vi "OwnCompat20261012_Native_GetRootDiagram.vi"() -> ()   [LabVIEW 2024]
panel:
  out "error out":errorcluster caption="错误输出"
  out "diagram_id":u32
  in  "diagram_id type":u32
  in  "target_path":path
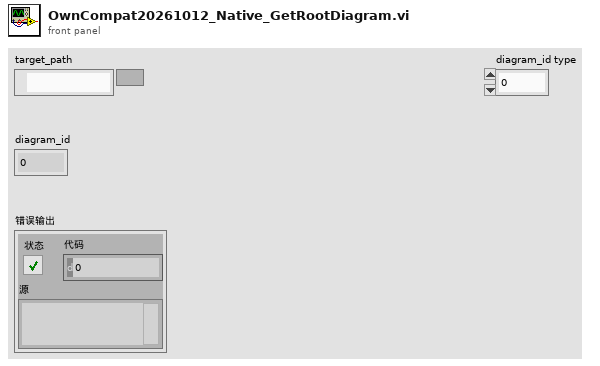
[diagram p1: front panel]
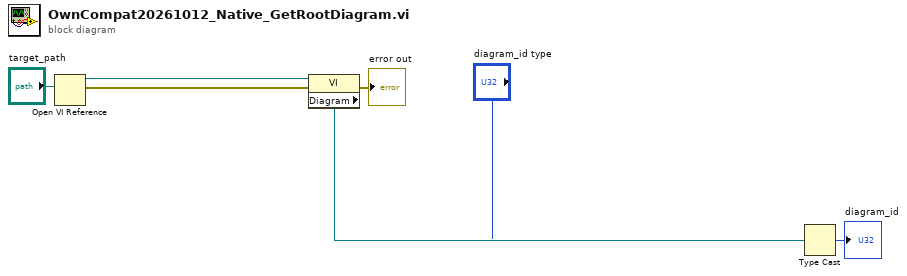
[diagram p0: block diagram]
diagram:
  n1 = Open VI Reference ("打开VI引用")(vi path="target_path") -> (vi reference=w6:refnum<vi>, error out=w5:errorcluster)  [unwired: 5 in]
  n2 = property on="属性节点" class="VI"(reference=w6, error in=w5) -> (error out=→"error out":errorcluster, "Diagram"=w4:refnum<vi>)  [unwired: 1 out]
  n3 = Type Cast ("强制类型转换")(type="diagram_id type", x=w4) -> (*(type *) &x=→"diagram_id":u32)
